vi "HandShaking.vi"(6 "Elapsed Time":u32, 8 "error in (no error)":errorcluster, 9 "Sequence Context":refnum<k7>, 10 "Stop":refnum<user-event>, 11 "OPC UA in":refnum<class "Abstract.lvclass">) -> (0 "error out":errorcluster, 3 "OPC UA out":refnum<class "Abstract.lvclass">)   [LabVIEW 2025, in "Abstract.lvclass"]
uses:
  Abstract.lvclass
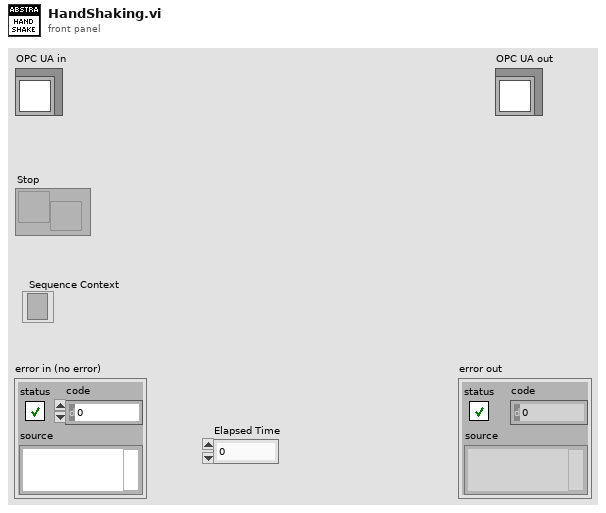
[diagram p1: front panel]
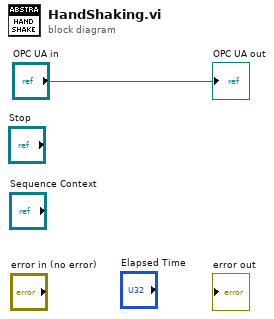
[diagram p0: block diagram]
diagram:
  "OPC UA out" <- "OPC UA in"
